vi "Save BMP File.vi"(4 "lpvBits Array":u8[](array[numeric]), 6 "Height":i32, 7 "Path to BMP file":path, 8 "error in":errorcluster, 9 "Width":i32, 10 "hbm":u32, 11 "hdc":u32) -> (0 "error out":errorcluster, 3 "Save Image Successful?":bool)   [LabVIEW 2025, in "Screenshot Utility.lvlib"]
uses:
  Screenshot Utility.lvlib
  <vilib>/picture/picture.llb/imagedata.ctl
  GDI32.DLL
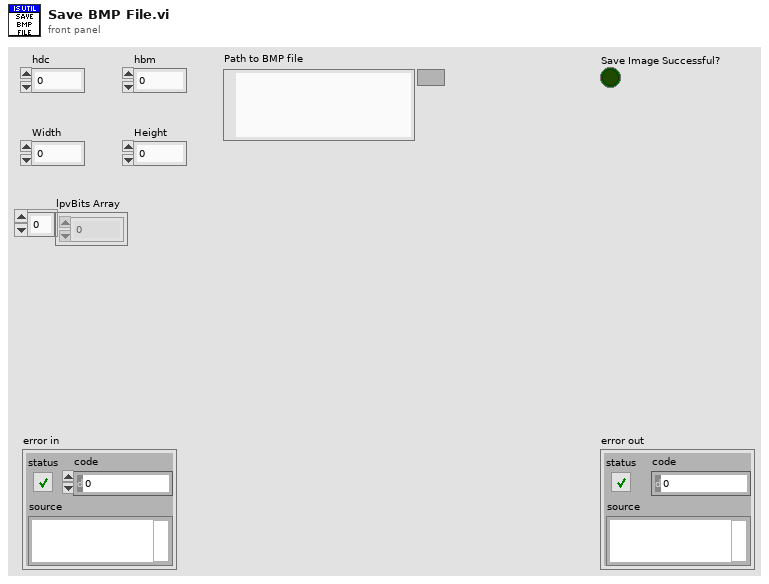
[diagram p1: front panel]
types:
  T1 = typedef "imagedata.ctl" = cluster{"image type":i32, "image depth":i32, "image":u8[], "mask":u8[], "colors":u32[], "Rectangle":cluster{"left":i16, "top":i16, "right":i16, "bottom":i16}}
  T2 = cluster{"biSize":u32, "biWidth":i32, "biHeight":i32, "biPlanes":u16, "biBitCount":u16, "biCompression":u32, "biSizeImage":u32, "biXPelsPerMeter":i32, "biYPelsPerMeter":i32, "biClrUsed":u32, "biClrImportant":u32}
  T3 = enum16{"big-endian, network order", "native, host order", "little-endian"}
  T4 = cluster{"left":i16, "top":i16, "right":i16, "bottom":i16}
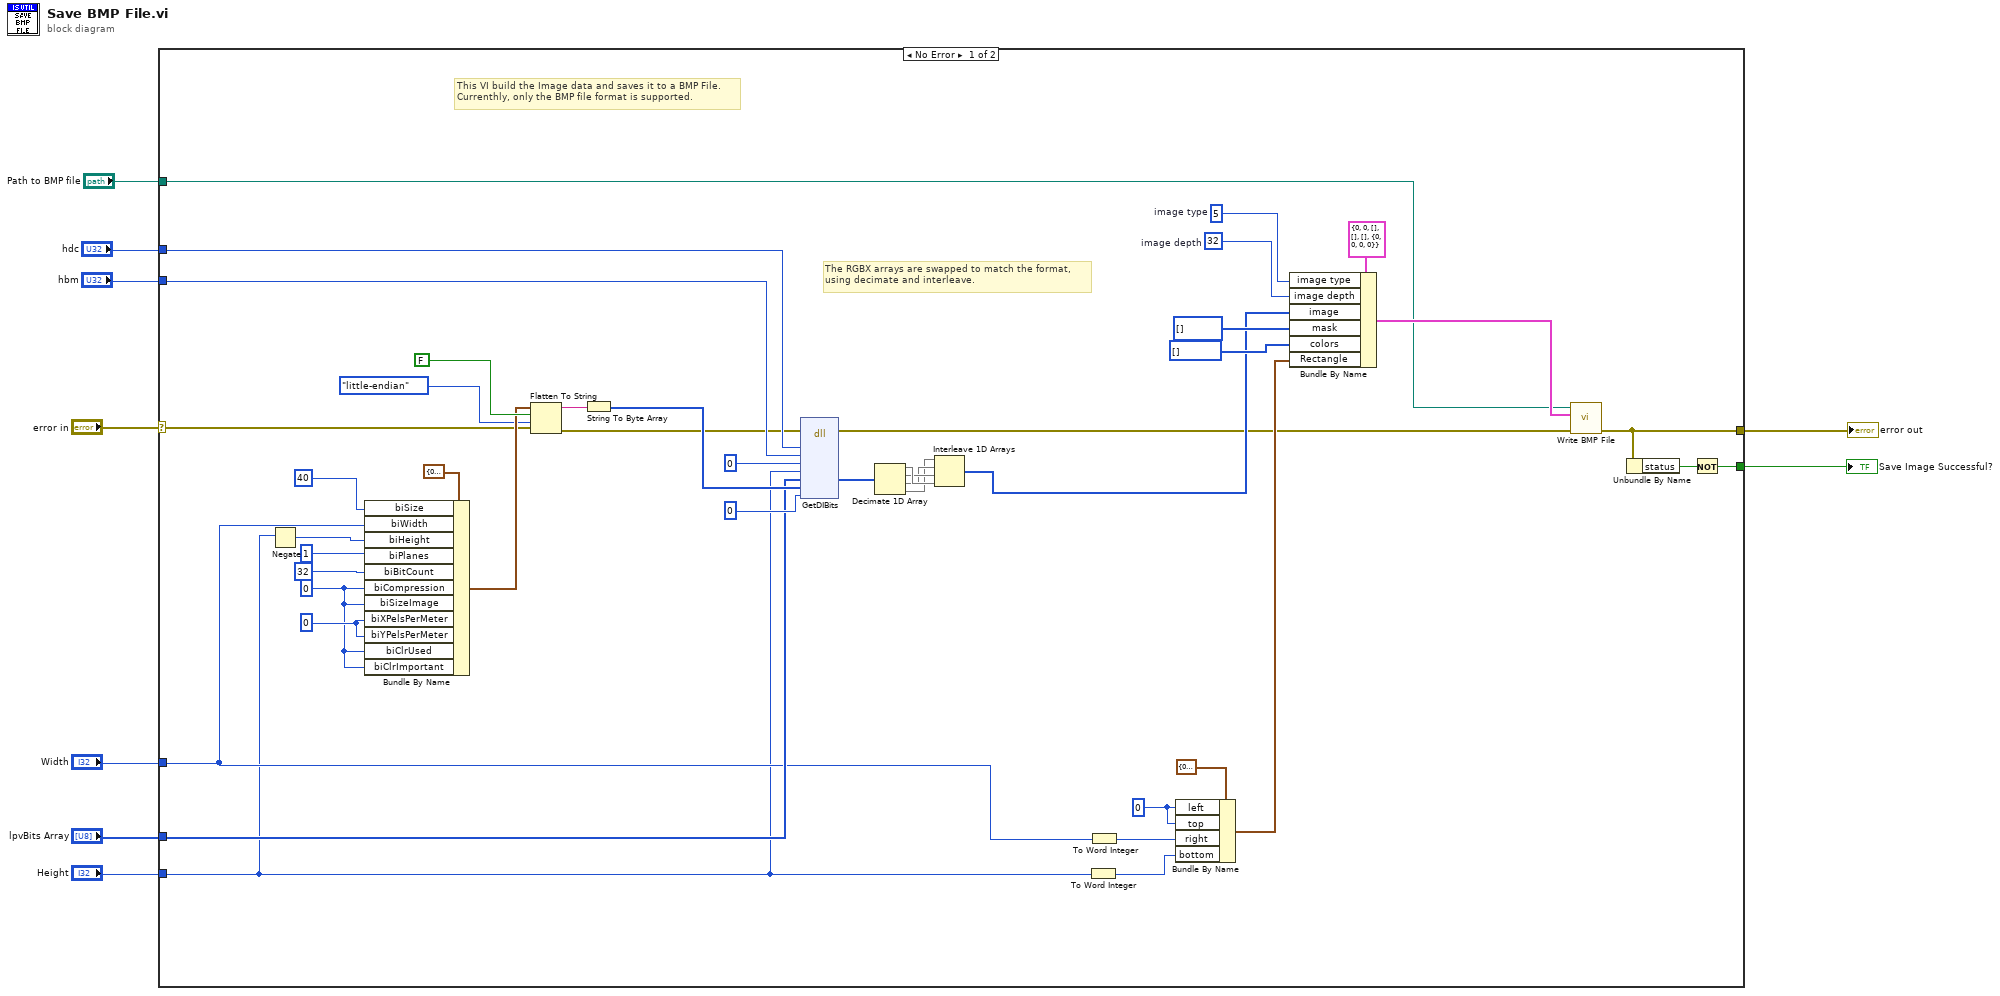
[diagram p0: block diagram]
diagram:
  n1 = case shown="No Error" "error in" {
    selector: "error in" -> [w20 w53]
    tunnel: "hbm" -> [w52 _]
    tunnel: "Width" -> [w14 _]
    tunnel: "Path to BMP file" -> [w10 _]
    tunnel: "hdc" -> [w29 _]
    tunnel: [w17 w53] -> w5
    tunnel: "lpvBits Array" -> [w19 _]
    tunnel: "Height" -> [w13 _]
    tunnel: [w15 _] -> w1
    frame No Error {
      w44 = 32  # image depth
      w43 = 5  # image type
      w33 = 0 ("biPlanes")
      w32 = u32 0 ("biPlanes")
      w27 = i16 0 ("left")
      # "The RGBX arrays are swapped to match the format,\nusing decimate and interleave."
      # "This VI build the Image data and saves it to a BMP File.\nCurrenthly, only the BMP file format is supported."
      n2 = Negate(x=w13) -> (-x=w36:i32)
      n3 = Bundle By Name(cluster=T2 {"biSize"=0, "biWidth"=0, "biHeight"=0, "biPlanes"=0, "biBitCount"=0, "biCompression"=0, "biSizeImage"=0, "biXPelsPerMeter"=0, "biYPelsPerMeter"=0, "biClrUsed"=0, "biClrImportant"=0}, "biSize"=u32 40, "biWidth"=w14, "biHeight"=w36, "biPlanes"=u16 1, "biBitCount"=u16 32, "biCompression"=w32, "biSizeImage"=w32, "biXPelsPerMeter"=w33, "biYPelsPerMeter"=w33, "biClrUsed"=w32, "biClrImportant"=w32) -> (w39:T2)
      n4 = Flatten To String(anything=w39, prepend array or string size? (T)=FALSE, byte order (0:big-endian, network order)=T3."little-endian", error in (no error)=w20) -> (data string=w22:string, error out=w21:errorcluster)  [unwired: 1 out]
      n5 = String To Byte Array(string=w22) -> (unsigned byte array=w40:u8[])
      n6 = dll-call lib="GDI32.DLL" fn="GetDIBits"(error in=w21, "hdc"=w29, "hbm"=w52, "start"=u32 0, "cLines"=w13, "lpvBits"=w19, "lpbmi"=w40, "usage"=u32 0) -> (error out=w11:errorcluster, "lpvBits"=w24:u8[])  [unwired: 2 in, 8 out]
      n7 = Decimate 1D Array(w24) -> (w51:u8[], w50:u8[], w49:u8[], w48:u8[])
      n8 = Interleave 1D Arrays(w48, w49, w50, w51) -> (w12:u8[])
      n9 = To Word Integer(number=w13) -> (16bit integer=w31:i16)
      n10 = To Word Integer(number=w14) -> (16bit integer=w30:i16)
      n11 = Bundle By Name(cluster=T4 {"left"=0, "top"=0, "right"=0, "bottom"=0} ("Rectangle"), "left"=w27, "top"=w27, "right"=w30, "bottom"=w31) -> (w26:T4)
      n12 = Bundle By Name(cluster=T1 {"image type"=0, "image depth"=0, "image"=[], "mask"=[], "colors"=[], "Rectangle"={"left"=0, "top"=0, "right"=0, "bottom"=0}} ("image data"), "image type"=w43, "image depth"=w44, "image"=w12, "mask"=u8[] [], "colors"=u32[] [], "Rectangle"=w26) -> (w47:T1)
      n13 = call <vilib>:"Write BMP File.vi"("error in (no error)"=w11, "image data"=w47, "path to BMP file"=w10) -> ("error out"=w17:errorcluster)  [unwired: 7 in, 1 out]
      n14 = Unbundle By Name(w17) -> ("status"=w16:bool)
      n15 = Not(x=w16) -> (.not. x?=w15:bool)
    }
    frame Error {
    }
  }
  "error out" <- w5
  "Save Image Successful?" <- w1
